vi "FuncVI-FileGetAppPath.vi"(5 "InstanceRef":T2, 9 "arg list":T1[](array[typedef]) {"num" format="%.2f"}) -> (0 "error out":bool, 3 "result":T1 {"num" format="%.2f"})   [LabVIEW 2021]
doc: "::: CalcExpress Toolkit :::\nCopyright (c) 2000-2026 Konstantin Shifershteyn. All rights reserved."
uses:
  cetypes.llb/CalcExpress Function Argument Info.ctl
  cetypes.llb/CalcExpress Instance RefNum.ctl
  cemisc.llb/[ce] CE component paths - Kind of Path Enum.ctl
panel:
  in  "max arg num":i32=1
  in  "min arg num":i32
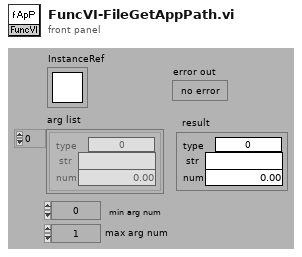
[diagram p1: front panel]
types:
  T1 = typedef "CalcExpress Function Argument Info.ctl" = cluster{"type":u32, "str":string, "num":dbl}
  T2 = typedef "CalcExpress Instance RefNum.ctl" = refnum<k1>
  T3 = cluster{"index":i32, "data type":enum32{"String", "DBL Number", "identifier", "1D Array of DBL", "2D Array of DBL", "CDB Number", "1D Array of CDB", "2D Array of CDB", "1D Array of String", "2D Array of String", "Unknown data type"}, "default num":dbl, "default str":string}[]
  T4 = enum32{"String", "DBL Number", "identifier", "1D Array of DBL", "2D Array of DBL", "CDB Number", "1D Array of CDB", "2D Array of CDB", "1D Array of String", "2D Array of String", "Unknown data type"}
  T5 = typedef "[ce] CE component paths - Kind of Path Enum.ctl" = enum16{"VIs", "FuncVIs", "Help", "Examples", "Project", "Templates"}
  T6 = cluster{"type: use this constant to specify a predefined type code":enum32{"String", "DBL Number", "identifier", "1D Array of DBL", "2D Array of DBL", "CDB Number", "1D Array of CDB", "2D Array of CDB", "1D Array of String", "2D Array of String", "Unknown data type"}, string, dbl}
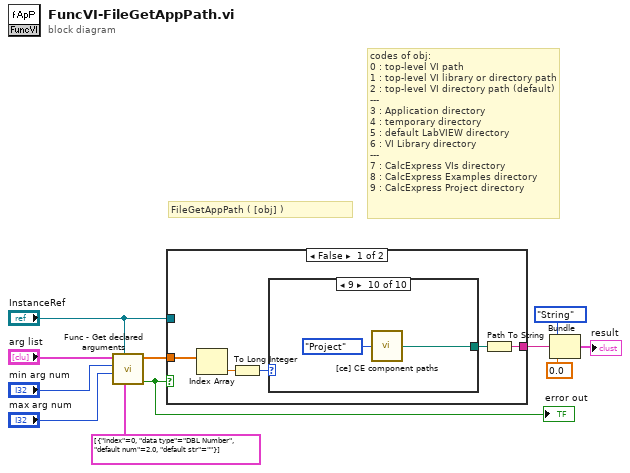
[diagram p0: block diagram]
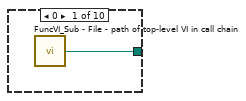
[diagram p2: hidden frame]
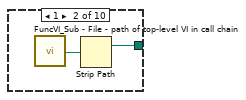
[diagram p3: hidden frame]
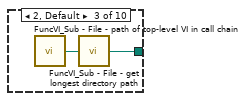
[diagram p4: hidden frame]
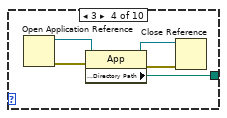
[diagram p5: hidden frame]
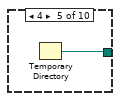
[diagram p6: hidden frame]
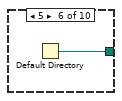
[diagram p7: hidden frame]
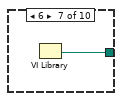
[diagram p8: hidden frame]
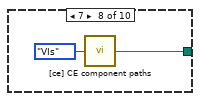
[diagram p9: hidden frame]
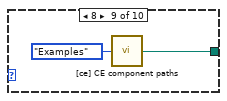
[diagram p10: hidden frame]
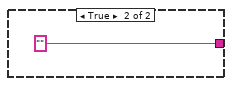
[diagram p11: hidden frame]
diagram:
  # "codes of obj:\n0 : top-level VI path\n1 : top-level VI library or directory path\n2 : top-level VI directory path (default)\n---\n3 : Application directory\n4 : temporary directory\n5 : default LabVIEW directory\n6 : VI Library directory\n---\n7 : CalcExpress VIs directory\n8 : CalcExpress Examples directory\n9 : CalcExpress Project directory"
  # "FileGetAppPath ( [obj] )"
  n1 = call "Func - Get declared arguments.vi"("arg descriptors"=T3 [{"index"=0, "data type"=enum."DBL Number", "default num"=2.0, "default str"=""}], "InstanceRef"="InstanceRef", "max arg num"="max arg num", "min arg num"="min arg num", "arg list"="arg list") -> ("error out"=w3:bool, "num list"=w5:dbl[])  [unwired: 3 in, 2 out]
  "error out" <- w3
  n2 = case shown="False" w3 {
    tunnel: "InstanceRef" -> [_ _]
    tunnel: w5 -> [w16 _]
    tunnel: [w12 ""] -> w4
    frame False {
      n3 = Index Array(array=w16) -> (element=w15:dbl)  [unwired: 1 in]
      n4 = To Long Integer(number=w15) -> (32bit integer=w14:i32)
      n5 = case shown="9" w14 {
        tunnel: [w17 w19 w21 w22 w27 w28 w29 w31 w33 w35] -> w13
        frame 0 {
          n6 = call "FuncVI_Sub - File - path of top-level VI in call chain.vi"() -> ("Top-Level VI Path"=w17:path)
        }
        frame 1 {
          n7 = call "FuncVI_Sub - File - path of top-level VI in call chain.vi"() -> ("Top-Level VI Path"=w18:path)
          n8 = Strip Path(path=w18) -> (stripped path=w19:path)  [unwired: 1 out]
        }
        frame 2, Default {
          n9 = call "FuncVI_Sub - File - path of top-level VI in call chain.vi"() -> ("Top-Level VI Path"=w20:path)
          n10 = call "FuncVI_Sub - File - get longest directory path.vi"("path in"=w20) -> ("path out"=w21:path)  [unwired: 4 in]
        }
        frame 3 {
          n11 = Open Application Reference() -> (0:w23:errorcluster, 3:w26:refnum<vi>)  [unwired: 4 in]
          n12 = property class="App"(reference=w26, error in=w23) -> (reference out=w25:refnum<vi>, error out=w24:errorcluster, "Application:Directory Path"=w22:path)
          n13 = Close Reference(reference=w25, error in (no error)=w24) -> ()  [unwired: 1 out]
        }
        frame 4 {
          n14 = Temporary Directory() -> (w27:path)
        }
        frame 5 {
          n15 = Default Directory() -> (w28:path)
        }
        frame 6 {
          n16 = VI Library() -> (path=w29:path)
        }
        frame 7 {
          n17 = call "[ce] CE component paths.vi"("kind of path"=[ce]_CE_component_paths_-_Kind_of_Path_Enum."VIs") -> ("path out"=w31:path)  [unwired: 1 in]
        }
        frame 8 {
          n18 = call "[ce] CE component paths.vi"("kind of path"=[ce]_CE_component_paths_-_Kind_of_Path_Enum."Examples") -> ("path out"=w33:path)  [unwired: 1 in]
        }
        frame 9 {
          n19 = call "[ce] CE component paths.vi"("kind of path"=[ce]_CE_component_paths_-_Kind_of_Path_Enum."Project") -> ("path out"=w35:path)  [unwired: 1 in]
        }
      }
      n20 = Path To String(path=w13) -> (string=w12:string)
    }
    frame True {
    }
  }
  n21 = Bundle("type: use this constant to specify a predefined type code"=T4."String", w4, 0.0) -> (→"result":T6)  [unwired: 1 in]
